vi "DPI Initialization.vi"(11 "DPE Project File Path":string) -> (0 "error out":errorcluster, 3 "DPI Instrument Name":refnum<k15>)   [LabVIEW 2025, in "Digital Pattern Sequencer.lvclass"]
uses:
  Digital Pattern Sequencer.lvclass
  Digital Pattern Sequencer.lvclass/Digital Pattern Sequencer.ctl
  <instrlib>/niDigital/niDigital.llb/niDigital Load Specifications Levels and Timing (Single).vi
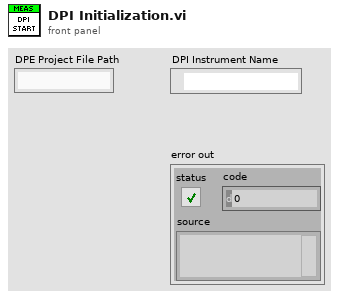
[diagram p1: front panel]
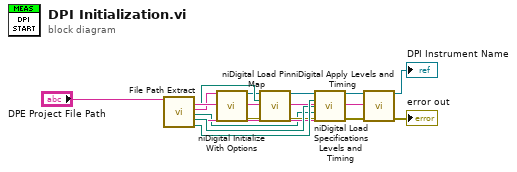
[diagram p0: block diagram]
diagram:
  n1 = call "File Path Extract.vi"("DPE Project File Path"="DPE Project File Path") -> ("Timing path name"=w10:string, "Level path name"=w11:string, ".pinmap file path"=w8:path, "DPI Instrument Name"=w9:string, ".digitiming file path"=w1:path, ".digilevels file path"=w12:path, ".spec file path"=w13:path)  [unwired: 10 in, 2 out]
  n2 = call <instrlib>:"niDigital Initialize With Options.vi"("resource name"=w9) -> ("instrument handle"=w6:refnum<k15>, "error out"=w7:errorcluster)  [unwired: 13 in]
  n3 = call <instrlib>:"niDigital Load Pin Map.vi"("instrument handle"=w6, "pin map file"=w8, "error in"=w7) -> ("instrument handle out"=w5:refnum<k15>, "error out"=w4:errorcluster)  [unwired: 11 in]
  n4 = call-poly <instrlib>:"niDigital Load Specifications Levels and Timing.vi"("instrument handle"=w5, "specifications file path"=w13, "levels file path"=w12, "timing file path"=w1, "error in"=w4) -> ("instrument handle out"=w16:refnum<k15>, "error out"=w15:errorcluster)  [unwired: 9 in]
  n5 = call <instrlib>:"niDigital Apply Levels and Timing.vi"("instrument handle"=w16, "levels sheet"=w11, "timing sheet"=w10, "error in"=w15) -> ("instrument handle out"=→"DPI Instrument Name":refnum<k15>, "error out"=→"error out":errorcluster)  [unwired: 10 in]
